vi "ASD Burst Reigon VI.vi"(8 "MAX Duration time(s)":dbl=0.02 format="%#_13g", 9 "R S IDX":i32[](array[numeric]), 10 "I underD0.01s":dbl[](array[numeric]), 11 "SDS":dbl[](array[numeric])) -> (0 "Burst Array":T1, 1 "Burst A":cluster{"Total Burst (s)":dbl, "B time (%)":dbl}, 2 "Burst Region (n)":i32, 3 "Burst Profile":cluster{i32[], "SDS":dbl[]}[](graph))   [LabVIEW 2018]
panel:
  out "x+y":i32[](array[numeric])
  out "配列 2":i32[](array[numeric])
  out "配列":i32[](array[numeric])
  out "S BRE IDX":i32[](array[numeric])
  out "S BRS IDX":i32[](array[numeric])
  out "サイズ":i32
  out "S Table":string[][](table) caption="B Table"
  out "B Time (%)":dbl
  out "Total Burst (ms)":dbl
  out "Burst time length":dbl[](array[numeric])
  out "Each Burst R#":i32[](array[numeric])
  out "BRStart IDX":i32[](array[numeric])
  out "BREnd IDX":i32[](array[numeric])
  out "REnd time":dbl[](array[numeric])
  out "RStart time":dbl[](array[numeric])
  out "x - y":i32
  out "Signal Peak END <0.01":dbl[](array[numeric])
  out "Signal Peak Start <0.01":dbl[](array[numeric])
  out "波形グラフ":dbl[](graph)
  out "Signal Duration between Peaks":dbl[](array[numeric])
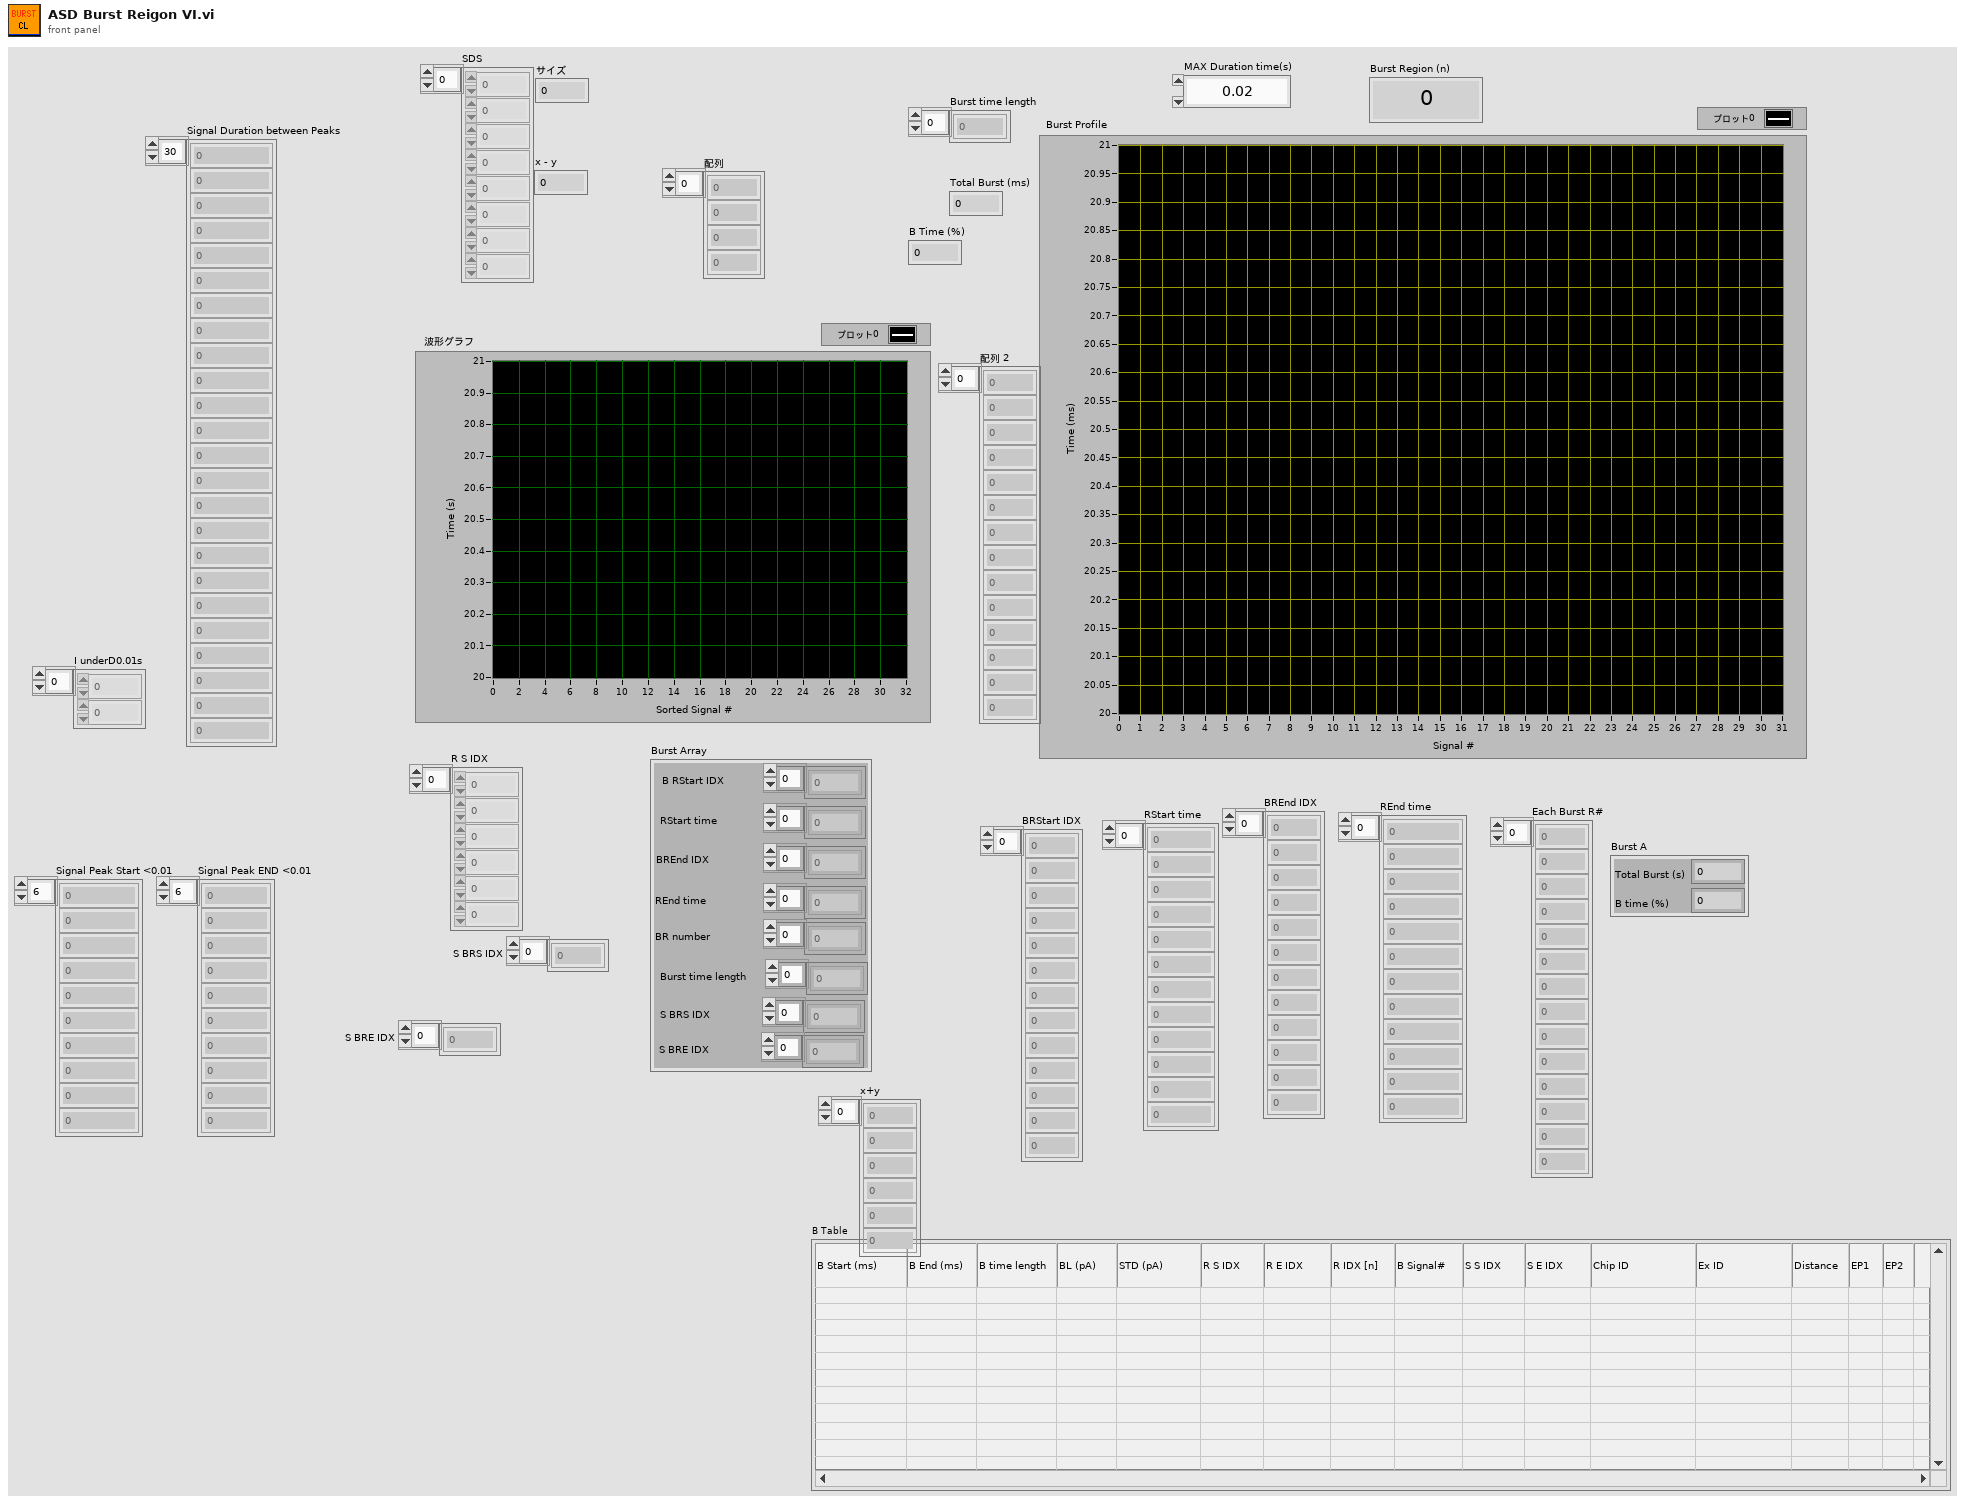
[diagram p1: front panel]
types:
  T1 = cluster{"B RStart IDX":i32[], "RStart time":dbl[], "BREnd IDX":i32[], "REnd time":dbl[], "BR number":dbl[], "Burst time length":dbl[], "S BRS IDX":i32[], "S BRE IDX":i32[]}
  T2 = cluster{i32[], dbl[], i32[], dbl[], i32[], dbl[], i32[], i32[]}
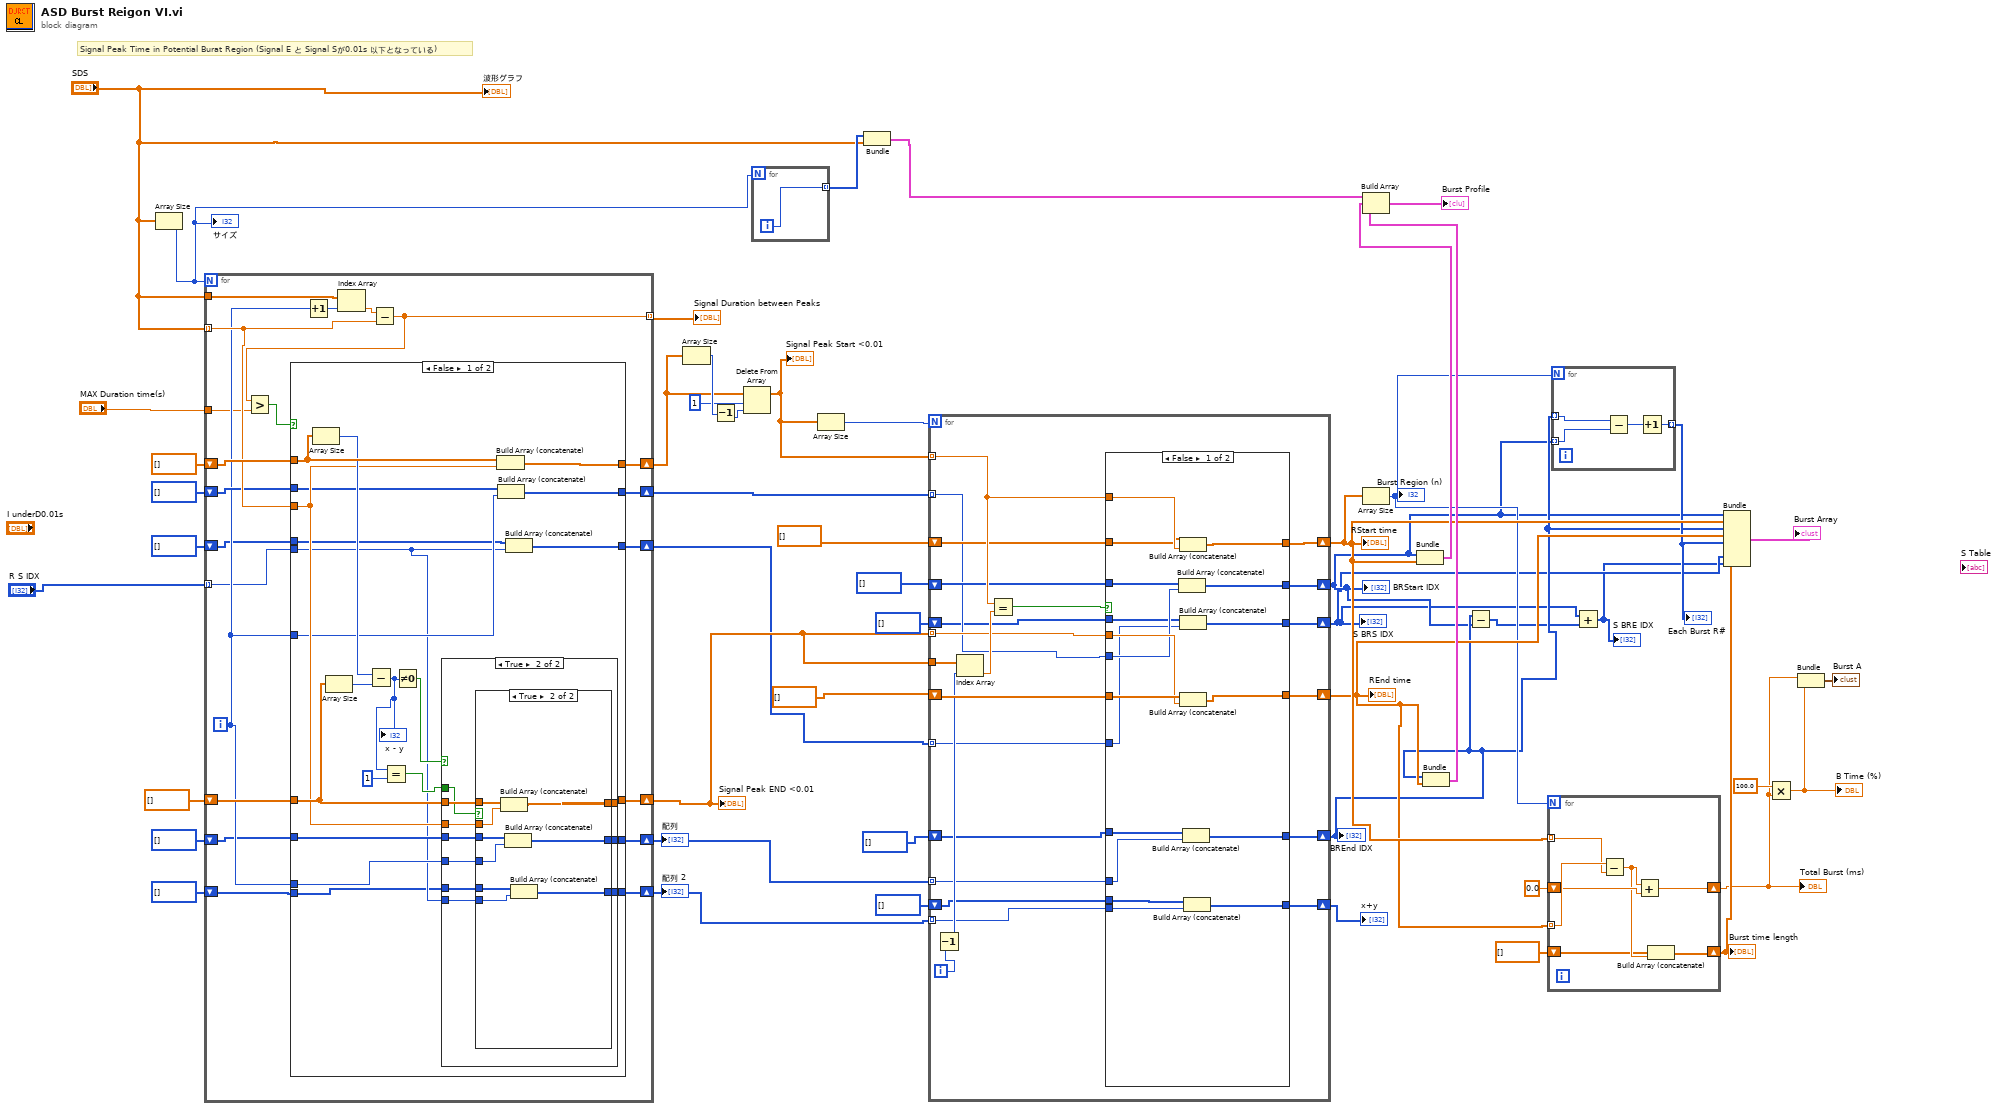
[diagram p0: block diagram]
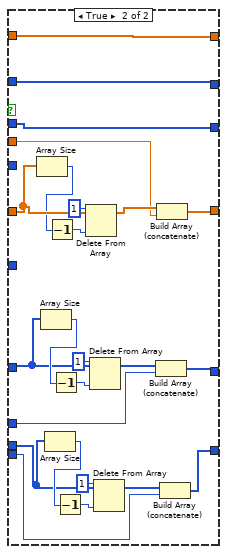
[diagram p2: hidden frame]
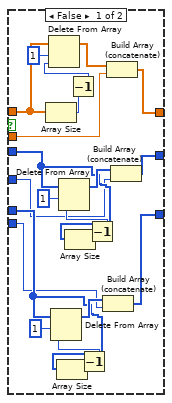
[diagram p4: hidden frame]
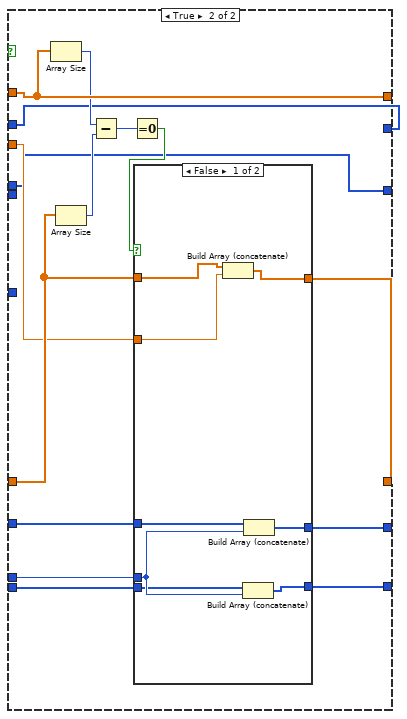
[diagram p5: hidden frame]
diagram:
  # "Signal Peak Time in Potential Burat Region (Signal E と Signal Sが0.01s 以下となっている)"
  n1 = Array Size(array="SDS") -> (size(s)=w39:i32)
  "サイズ" <- w39
  n2 = for {
    N: w39 -> [_]
    tunnel: "SDS" -> [w70]
    tunnel: "SDS" -> [w63] mode=indexing
    tunnel: [w69] -> w51 mode=indexing
    shift-right: [w67] -> w45
    shift-left: dbl[] [] -> [w66]
    shift-right: [w64] -> w42
    shift-left: dbl[] [] -> [w65]
    shift-right: [w62] -> w36
    shift-left: i32[] [] -> [w61]
    shift-right: [w59] -> w32
    shift-left: i32[] [] -> [w58]
    tunnel: "MAX Duration time(s)" -> [w57]
    tunnel: "R S IDX" -> [w56] mode=indexing
    shift-right: [w55] -> w11
    shift-left: i32[] [] -> [w54]
    shift-right: [w53] -> w8
    shift-left: i32[] [] -> [w52]
    i -> [w60]
    n3 = Increment(x=w60) -> (x+1=w71:i32)
    n4 = Index Array(array=w70, index=w71) -> (element=w72:dbl)
    n5 = Subtract(x=w72, y=w63) -> (x-y=w69:dbl)
    n6 = Greater?(x=w69, y=w57) -> (0:w68:bool)
    n7 = case shown="False" w68 {
      tunnel: [w94 w152] -> w67
      tunnel: w66 -> [w92 w152]
      tunnel: w65 -> [w85 w147]
      tunnel: [w93 w146] -> w64
      tunnel: w63 -> [w84 w145]
      tunnel: w60 -> [w83 _]
      tunnel: [w82 w144] -> w62
      tunnel: w61 -> [w81 w144]
      tunnel: w60 -> [w80 w142]
      tunnel: [w79 w141] -> w59
      tunnel: w58 -> [w78 w143]
      tunnel: w56 -> [w75 _]
      tunnel: [w77 w140] -> w55
      tunnel: w54 -> [w76 w140]
      tunnel: [w74 w139] -> w53
      tunnel: w52 -> [w73 w138]
      frame False {
        n8 = Array Size(array=w92) -> (size(s)=w91:i32)
        n9 = Array Size(array=w85) -> (size(s)=w90:i32)
        n10 = Subtract(x=w91, y=w90) -> (x-y=w88:i32)
        "x - y" <- w88
        n11 = Equal?(x=w88, y=1) -> (x = y?=w86:bool)
        n12 = Not Equal To 0?(x=w88) -> (x != 0?=w89:bool)
        n13 = case shown="True" w89 {
          tunnel: w85 -> [w97 w107]
          tunnel: [w97 w106] -> w93
          tunnel: w84 -> [_ w105]
          tunnel: w86 -> [_ w104]
          tunnel: w80 -> [_ w103]
          tunnel: [w96 w102] -> w79
          tunnel: w78 -> [w96 w101]
          tunnel: w75 -> [_ w100]
          tunnel: [w95 w99] -> w74
          tunnel: w73 -> [w95 w98]
          frame False {
          }
          frame True {
            n14 = case shown="True" w104 {
              tunnel: w107 -> [w128 w137]
              tunnel: [w122 w136] -> w106
              tunnel: w105 -> [w123 w135]
              tunnel: w103 -> [w109 w134]
              tunnel: [w120 w133] -> w102
              tunnel: w101 -> [w118 w132]
              tunnel: w100 -> [w108 w131]
              tunnel: [w111 w130] -> w99
              tunnel: w98 -> [w110 w129]
              frame False {
                n15 = Array Size(array=w128) -> (size(s)=w127:i32)
                n16 = Array Size(array=w110) -> (size(s)=w113:i32)
                n17 = Array Size(array=w118) -> (size(s)=w117:i32)
                n18 = Decrement(x=w127) -> (x-1=w125:i32)
                n19 = Delete From Array(array=w128, length=1 ("長さ"), index=w125) -> (array with subset deleted=w124:dbl[])  [unwired: 1 out]
                n20 = Decrement(x=w113) -> (x-1=w112:i32)
                n21 = Delete From Array(array=w110, length=1 ("長さ"), index=w112) -> (array with subset deleted=w115:i32[])  [unwired: 1 out]
                n22 = Decrement(x=w117) -> (x-1=w116:i32)
                n23 = Delete From Array(array=w118, length=1 ("長さ"), index=w116) -> (array with subset deleted=w121:i32[])  [unwired: 1 out]
                n24 = Build Array (concatenate)(w115, w108) -> (w111:i32[])
                n25 = Build Array (concatenate)(w124, w123) -> (w122:dbl[])
                n26 = Build Array (concatenate)(w121, w109) -> (w120:i32[])
              }
              frame True {
                n27 = Build Array (concatenate)(w137, w135) -> (w136:dbl[])
                n28 = Build Array (concatenate)(w132, w134) -> (w133:i32[])
                n29 = Build Array (concatenate)(w129, w131) -> (w130:i32[])
              }
            }
          }
        }
        n30 = Build Array (concatenate)(w92, w84) -> (w94:dbl[])
        n31 = Build Array (concatenate)(w81, w83) -> (w82:i32[])
        n32 = Build Array (concatenate)(w76, w75) -> (w77:i32[])
      }
      frame True {
        n33 = Array Size(array=w152) -> (size(s)=w151:i32)
        n34 = Array Size(array=w147) -> (size(s)=w150:i32)
        n35 = Subtract(x=w151, y=w150) -> (x-y=w149:i32)
        n36 = Equal To 0?(x=w149) -> (x = 0?=w148:bool)
        n37 = case shown="False" w148 {
          tunnel: w147 -> [w160 w163]
          tunnel: [w159 w163] -> w146
          tunnel: w145 -> [w158 _]
          tunnel: w143 -> [w157 w162]
          tunnel: w142 -> [w155 _]
          tunnel: [w156 w162] -> w141
          tunnel: [w154 w161] -> w139
          tunnel: w138 -> [w153 w161]
          frame False {
            n38 = Build Array (concatenate)(w160, w158) -> (w159:dbl[])
            n39 = Build Array (concatenate)(w153, w155) -> (w154:i32[])
            n40 = Build Array (concatenate)(w157, w155) -> (w156:i32[])
          }
          frame True {
          }
        }
      }
    }
  }
  "Signal Duration between Peaks" <- w51
  "Signal Peak END <0.01" <- w42
  "配列" <- w32
  "配列 2" <- w8
  n41 = Array Size(array=w45) -> (size(s)=w48:i32)
  n42 = Decrement(x=w48) -> (x-1=w46:i32)
  n43 = Delete From Array(array=w45, length=1 ("長さ"), index=w46) -> (array with subset deleted=w43:dbl[])  [unwired: 1 out]
  "Signal Peak Start <0.01" <- w43
  n44 = for {
    N: w39 -> [_]
    tunnel: [w164] -> w38 mode=indexing
    i -> [w164]
  }
  n45 = Array Size(array=w43) -> (size(s)=w44:i32)
  n46 = Bundle(w38, "SDS"="SDS") -> (w31:cluster{i32[], "SDS":dbl[]})  [unwired: 1 in]
  n47 = for {
    N: w44 -> [_]
    tunnel: w43 -> [w180] mode=indexing
    tunnel: w42 -> [w181] mode=indexing
    tunnel: w42 -> [w187]
    shift-right: [w182] -> w23
    shift-left: dbl[] [] -> [w183]
    shift-right: [w179] -> w24
    shift-left: dbl[] [] -> [w178]
    tunnel: w36 -> [w173] mode=indexing
    tunnel: w32 -> [w171] mode=indexing
    shift-right: [w176] -> w5
    shift-left: i32[] [] -> [w177]
    shift-right: [w172] -> w6
    shift-left: i32[] [] -> [w174]
    tunnel: w11 -> [w170] mode=indexing
    shift-right: [w169] -> w2
    shift-left: i32[] [] -> [w168]
    tunnel: w8 -> [w167] mode=indexing
    shift-right: [w166] -> w3
    shift-left: i32[] [] -> [w165]
    i -> [w186]
    n48 = Decrement(x=w186) -> (x-1=w175:i32)
    n49 = Index Array(array=w187, index=w175) -> (element=w185:dbl)
    n50 = Equal?(x=w180, y=w185) -> (x = y?=w184:bool)
    n51 = case shown="False" w184 {
      tunnel: w183 -> [w205 w227]
      tunnel: [w204 w223] -> w182
      tunnel: w181 -> [w203 w222]
      tunnel: w180 -> [w202 _]
      tunnel: [w201 w225] -> w179
      tunnel: w178 -> [w200 w225]
      tunnel: w177 -> [w199 w221]
      tunnel: [w198 w221] -> w176
      tunnel: w173 -> [w197 _]
      tunnel: w174 -> [w196 w217]
      tunnel: [w195 w215] -> w172
      tunnel: w171 -> [w194 w207]
      tunnel: w170 -> [w193 _]
      tunnel: [w192 w214] -> w169
      tunnel: w168 -> [w191 w214]
      tunnel: w167 -> [w190 w206]
      tunnel: [w189 w208] -> w166
      tunnel: w165 -> [w188 w209]
      frame False {
        n52 = Build Array (concatenate)(w199, w197) -> (w198:i32[])
        n53 = Build Array (concatenate)(w200, w202) -> (w201:dbl[])
        n54 = Build Array (concatenate)(w205, w203) -> (w204:dbl[])
        n55 = Build Array (concatenate)(w191, w193) -> (w192:i32[])
        n56 = Build Array (concatenate)(w196, w194) -> (w195:i32[])
        n57 = Build Array (concatenate)(w188, w190) -> (w189:i32[])
      }
      frame True {
        n58 = Array Size(array=w227) -> (size(s)=w226:i32)
        n59 = Array Size(array=w217) -> (size(s)=w218:i32)
        n60 = Array Size(array=w209) -> (size(s)=w211:i32)
        n61 = Decrement(x=w226) -> (x-1=w229:i32)
        n62 = Decrement(x=w218) -> (x-1=w220:i32)
        n63 = Decrement(x=w211) -> (x-1=w213:i32)
        n64 = Delete From Array(array=w227, length=1 ("長さ"), index=w229) -> (array with subset deleted=w224:dbl[])  [unwired: 1 out]
        n65 = Delete From Array(array=w217, length=1 ("長さ"), index=w220) -> (array with subset deleted=w216:i32[])  [unwired: 1 out]
        n66 = Delete From Array(array=w209, length=1 ("長さ"), index=w213) -> (array with subset deleted=w210:i32[])  [unwired: 1 out]
        n67 = Build Array (concatenate)(w216, w207) -> (w215:i32[])
        n68 = Build Array (concatenate)(w224, w222) -> (w223:dbl[])
        n69 = Build Array (concatenate)(w210, w206) -> (w208:i32[])
      }
    }
  }
  "RStart time" <- w24
  "REnd time" <- w23
  "BREnd IDX" <- w6
  "BRStart IDX" <- w5
  "S BRS IDX" <- w2
  "x+y" <- w3
  n70 = Array Size(array=w24) -> (size(s)=w15:i32)
  "Burst Region (n)" <- w15
  n71 = Bundle(w5, w24) -> (w30:cluster{i32[], dbl[]})  [unwired: 1 in]
  n72 = Bundle(w6, w23) -> (w29:cluster{i32[], dbl[]})  [unwired: 1 in]
  n73 = Build Array(w31, w30, w29) -> (→"Burst Profile":cluster{i32[], "SDS":dbl[]}[])
  n74 = Subtract(x=w6, y=w5) -> (x-y=w4:i32[])
  n75 = for {
    N: w15 -> [_]
    tunnel: w24 -> [w235] mode=indexing
    tunnel: w23 -> [w236] mode=indexing
    shift-right: [w233] -> w18
    shift-left: 0.0 -> [w234]
    shift-right: [w231] -> w19
    shift-left: dbl[] [] -> [w230]
    n76 = Subtract(x=w236, y=w235) -> (x-y=w232:dbl)
    n77 = Add(x=w232, y=w234) -> (x+y=w233:dbl)
    n78 = Build Array (concatenate)(w230, w232) -> (w231:dbl[])
  }
  "Burst time length" <- w19
  "Total Burst (ms)" <- w18
  n79 = for {
    N: w15 -> [_]
    tunnel: w6 -> [w240] mode=indexing
    tunnel: w5 -> [w239] mode=indexing
    tunnel: [w237] -> w14 mode=indexing
    n80 = Subtract(x=w240, y=w239) -> (x-y=w238:i32)
    n81 = Increment(x=w238) -> (x+1=w237:i32)
  }
  "Each Burst R#" <- w14
  n82 = Add(x=w2, y=w4) -> (x+y=w1:i32[])
  "S BRE IDX" <- w1
  n83 = Bundle(w5, w24, w6, w23, w14, w19, w2, w1) -> (→"Burst Array":T2)  [unwired: 1 in]
  n84 = Multiply(x=100.0, y=w18) -> (x*y=w17:dbl)
  "B Time (%)" <- w17
  n85 = Bundle(w18, w17) -> (→"Burst A":cluster{dbl, dbl})  [unwired: 1 in]
  "波形グラフ" <- "SDS"
